vi "Get Message.vi"(8 "error in (no error)":errorcluster, 11 "SPARC4_GUI in":refnum<class "SPARC4_GEI.lvclass">) -> (0 "error out":errorcluster, 3 "SPARC4_GUI out":refnum<class "SPARC4_GEI.lvclass">)   [LabVIEW 2018, in "SPARC4_GEI.lvclass"]
uses:
  SPARC4_GEI.lvclass
  Channel GUI/Channel.lvclass
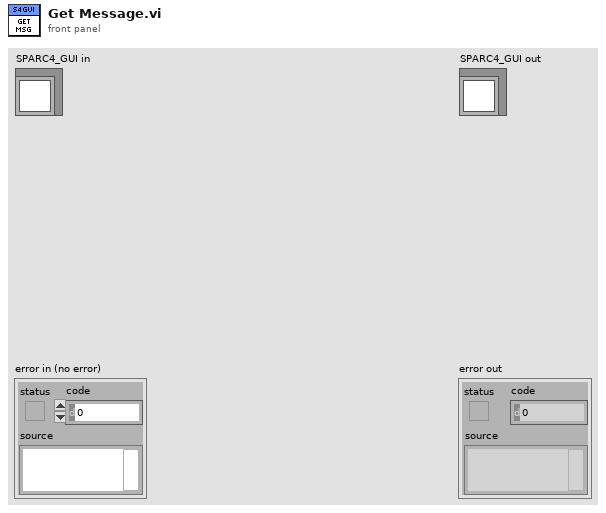
[diagram p1: front panel]
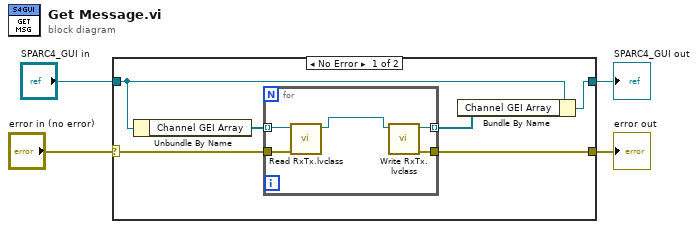
[diagram p0: block diagram]
diagram:
  n1 = case shown="No Error" "error in (no error)" {
    selector: "error in (no error)" -> [w6 w17]
    tunnel: [w8 w17] -> w3
    tunnel: [w9 w16] -> w1
    tunnel: "SPARC4_GUI in" -> [w10 w16]
    frame No Error {
      n2 = Unbundle By Name(w10) -> ("Channel GEI Array"=w7:refnum<class "Channel GEI.lvclass">[])
      n3 = for {
        tunnel: [w11] -> w8
        tunnel: w7 -> [w14] mode=indexing
        tunnel: w6 -> [w13]
        tunnel: [w12] -> w5 mode=indexing
        n4 = call "Read RxTx.lvclass.vi"("error in (no error)"=w13, "Channel GUI in"=w14) -> ("Channel GUI out"=w15:refnum<class "Channel.lvclass">)  [unwired: 7 in, 2 out]
        n5 = call "Write RxTx.lvclass.vi"("Channel GUI in"=w15) -> ("error out"=w11:errorcluster, "Channel GUI out"=w12:refnum<class "Channel.lvclass">)  [unwired: 9 in]
      }
      n6 = Bundle By Name(cluster=w10, "Channel GEI Array"=w5) -> (w9:refnum<class "SPARC4_GEI.lvclass">)
    }
    frame Error {
    }
  }
  "error out" <- w3
  "SPARC4_GUI out" <- w1
